vi "libssh2_channel_process_startup.vi"(8 "error in (no error)":errorcluster, 9 "message":string, 10 "request":string, 11 "channel":T1) -> (0 "error out":errorcluster)   [LabVIEW 2017, in "libssh2.lvlib"]
doc: "Start a process on a channel."
uses:
  libssh2.lvlib
  Channel Refnum.ctl
  Acquire Session.vi
  Release Session.vi
  Not A Channel.vi
  <vilib>/Utility/error.llb/Error Cluster From Error Code.vi
  Global Settings.vi
  Read Channel Refnum.vi
  Read Session Refnum.vi
  <vilib>/Utility/semaphor.llb/Acquire Semaphore.vi
  <vilib>/Utility/semaphor.llb/Release Semaphore.vi
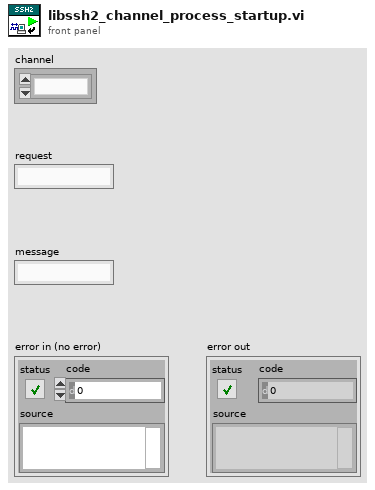
[diagram p1: front panel]
types:
  T1 = typedef "libssh2.lvlib/Channel Refnum.ctl" = refnum<k1>
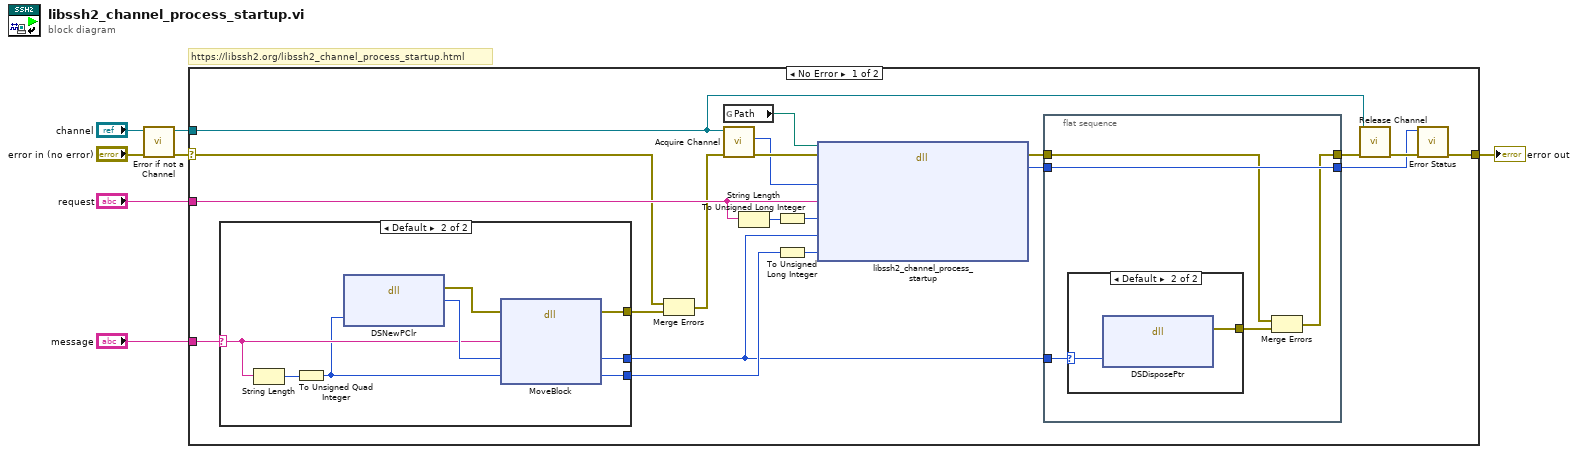
[diagram p0: block diagram]
diagram:
  # "https://libssh2.org/libssh2_channel_process_startup.html"
  n1 = call "Error if not a Channel.vi"("error in (no error)"="error in (no error)", "channel"="channel") -> ("error out"=w3:errorcluster, "channel out"=w1:T1)  [unwired: 8 in]
  n2 = case shown="No Error" w3 {
    selector: w3 -> [w26 w43]
    tunnel: "request" -> [w27 _]
    tunnel: "message" -> [w10 _]
    tunnel: [w25 w43] -> w5
    tunnel: w1 -> [w18 _]
    frame No Error {
      n3 = case shown="Default" w10 {
        selector: w10 -> [_ w29]
        tunnel: [_ w33] -> w16
        tunnel: [_ w32] -> w15
        tunnel: [_ w30] -> w8
        frame "" {
        }
        frame Default {
          n4 = String Length(string=w29) -> (length=w35:i32)
          n5 = To Unsigned Quad Integer(1:w35) -> (0:w28:u64)
          n6 = dll-call lib="LabVIEW" fn="DSNewPClr"("size"=w28) -> (error out=w31:errorcluster, "return type"=w34:u64)  [unwired: 4 in, 1 out]
          n7 = dll-call lib="LabVIEW" fn="MoveBlock"(error in=w31, "ps"=w29, "pd"=w34, "size"=w28) -> (error out=w30:errorcluster, "pd"=w32:u64, "size"=w33:u64)  [unwired: 4 in, 1 out]
        }
      }
      n8 = Merge Errors(w26, w8) -> (w9:errorcluster)
      n9 = global read "Global Settings.vi" "Path"() -> (w20:path)
      n10 = call "Acquire Channel.vi"("error in (no error)"=w9, "channel"=w18) -> ("error out"=w23:errorcluster, "LIBSSH2_CHANNEL*"=w22:u64)  [unwired: 8 in]
      n11 = String Length(string=w27) -> (length=w21:i32)
      n12 = To Unsigned Long Integer(number=w21) -> (unsigned 32bit integer=w24:u32)
      n13 = To Unsigned Long Integer(number=w16) -> (unsigned 32bit integer=w17:u32)
      n14 = dll-call lib="?" fn="libssh2_channel_process_startup"(path in=w20, error in=w23, "channel"=w22, "request"=w27, "request_len"=w24, "message"=w15, "message_len"=w17) -> (error out=w11:errorcluster, "return value"=w13:i32)  [unwired: 6 in, 1 out]
      n15 = flat-sequence {
        tunnel: w15 -> [w39]
        tunnel: [w40] -> w14
        tunnel: w13 -> [w40]
        tunnel: [w36] -> w12
        tunnel: w11 -> [w37]
        frame #0 {
          n16 = case shown="Default" w39 {
            selector: w39 -> [_ w42]
            tunnel: [_ w41] -> w38
            frame 0 {
            }
            frame Default {
              n17 = dll-call lib="LabVIEW" fn="DSDisposePtr"("p"=w42) -> (error out=w41:errorcluster)  [unwired: 5 in, 1 out]
            }
          }
          n18 = Merge Errors(w37, w38) -> (w36:errorcluster)
        }
      }
      n19 = call "Release Channel.vi"("error in (no error)"=w12, "channel"=w18) -> ("error out"=w19:errorcluster)  [unwired: 9 in]
      n20 = call "Error Status.vi"("error in (no error)"=w19, "return value"=w14) -> ("error out"=w25:errorcluster)  [unwired: 8 in, 1 out]
    }
    frame Error {
    }
  }
  "error out" <- w5
